vi "labview-quick-run.vi"   [LabVIEW 2020]
uses:
  User/User.lvclass
  Nominal Client/Nominal Client.lvclass
  nominal types/workspace/workspace.lvclass
  submodules/reqwest-labview/lv-src/reqwest/reqwest.lvclass
  e79185ee-863a-4b48-b269-365b27d9e424.vi
  Run/Run.lvclass
  asset/asset.lvclass
  Nominal Client/asset.get.vi
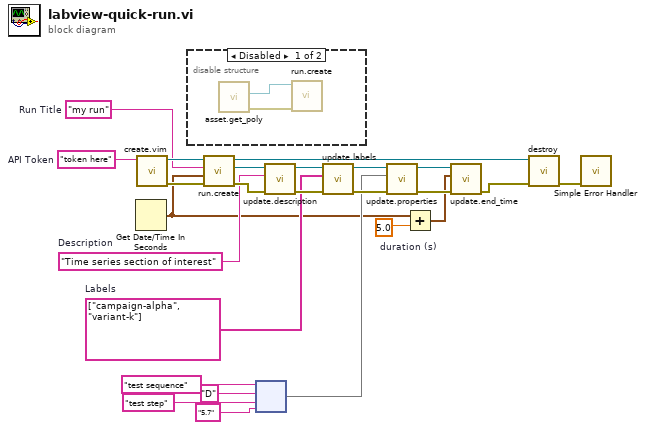
[diagram p0: block diagram]
diagram:
  w1 = 5.0  # duration (s)
  w11 = string[] ["campaign-alpha", "variant-k"]  # Labels
  w14 = "Time series section of interest"  # Description
  w24 = "token here"  # API Token
  w17 = "my run"  # Run Title
  n1 = Get Date/Time In Seconds() -> (seconds since 1Jan1904=w2:timestamp)
  n2 = call "create.vim"("API Token (string or path)"=w24) -> ("error out"=w18:errorcluster, "Nominal Client"=w19:refnum<class "Nominal Client.lvclass">)  [unwired: 8 in, 1 out]
  n3 = disable-structure shown="Disabled" {
    frame Disabled {
      n4 = call-poly "asset.get_poly.vi"() -> ("error out"=w26:errorcluster, "Asset"=w27:refnum<class "asset.lvclass">)  [unwired: 9 in, 1 out]
      n5 = call "run.create.vi"("error in"=w26, "asset in"=w27) -> ()  [unwired: 7 in, 3 out]
    }
    frame Enabled {
    }
  }
  n6 = call "run.create.vi"("error in"=w18, "Start Time (now)"=w2, "Title"=w17, "Nominal Client in"=w19) -> ("error out"=w15:errorcluster, "Run"=w16:refnum<class "Run.lvclass">, "Nominal Client out"=w8:refnum<class "Nominal Client.lvclass">)  [unwired: 5 in]
  n7 = node("test sequence", "D", "test step", "5.7") -> (w7:map{string, string})
  n8 = call "update.description.vi"("error in (no error)"=w15, "Description"=w14, "Run in"=w16) -> ("error out"=w12:errorcluster, "Run out"=w13:refnum<class "Run.lvclass">)  [unwired: 7 in]
  n9 = call "update.labels.vi"("error in (no error)"=w12, "labels"=w11, "Run in"=w13) -> ("error out"=w9:errorcluster, "Run out"=w10:refnum<class "Run.lvclass">)  [unwired: 7 in]
  n10 = call "update.properties.vi"("error in (no error)"=w9, "properties"=w7, "Run in"=w10) -> ("error out"=w6:errorcluster, "Run out"=w5:refnum<class "Run.lvclass">)  [unwired: 7 in]
  n11 = Add(x=w2, y=w1) -> (x+y=w3:timestamp)
  n12 = call "update.end_time.vi"("error in (no error)"=w6, "End Time (now)"=w3, "Run in"=w5) -> ("error out"=w4:errorcluster)  [unwired: 7 in, 1 out]
  n13 = call "destroy.vi"("error in"=w4, "Nominal Client"=w8) -> ("error out"=w25:errorcluster)  [unwired: 9 in]
  n14 = call <vilib>:"Simple Error Handler.vi"("error in (no error)"=w25) -> ()  [unwired: 4 in, 5 out]
